vi "set--uid--tags.vi"() -> ()   [LabVIEW 2021]
panel:
  out "Array 2":string[](array[string])
  out "Array":i32[](array[numeric])
  out "error out":errorcluster
  # "String"
  # "Digital"
  # "Multicolumn Listbox"
  # "Digital"
  # "Listbox"
  # "Ring"
  # "Table"
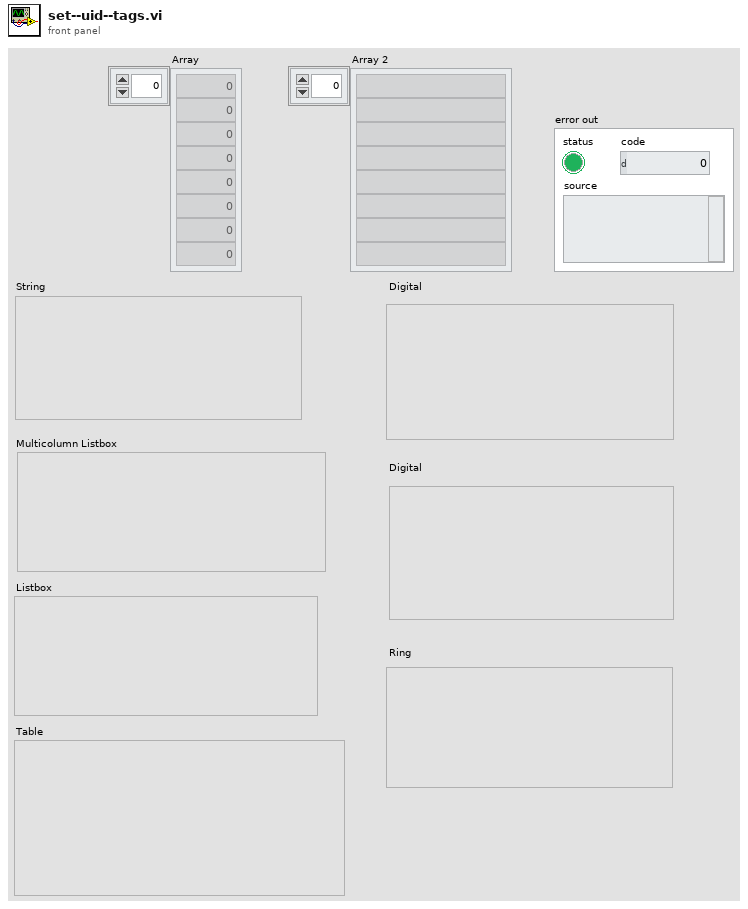
[diagram p1: front panel]
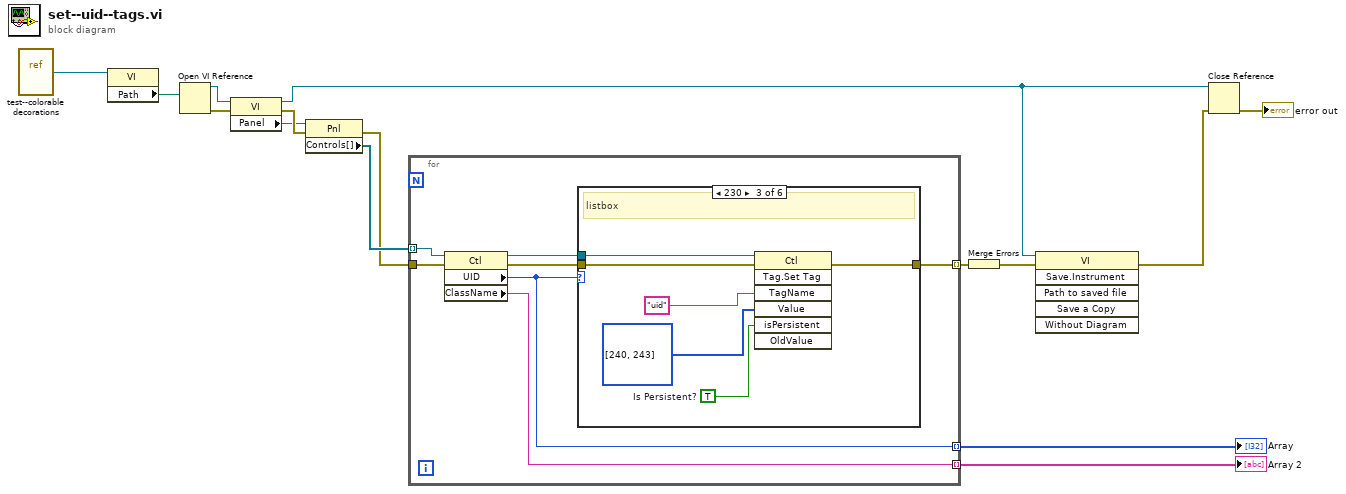
[diagram p0: block diagram]
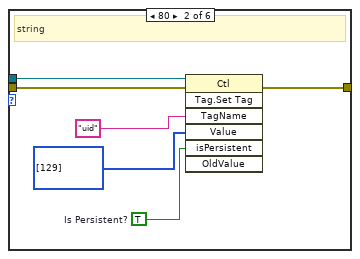
[diagram p3: hidden frame]
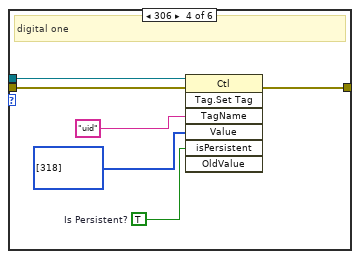
[diagram p4: hidden frame]
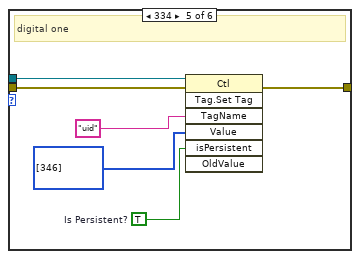
[diagram p5: hidden frame]
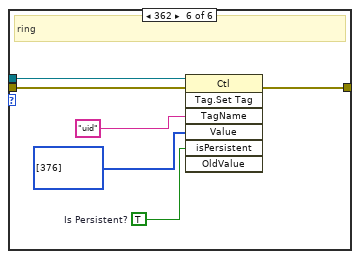
[diagram p6: hidden frame]
diagram:
  n1 = vi-ref "test--colorable decorations.vi"() -> (w15:refnum<vi>)
  n2 = property class="VI"(reference=w15) -> ("Path"=w12:path)  [unwired: 1 in, 2 out]
  n3 = Open VI Reference(vi path=w12) -> (vi reference=w10:refnum<vi>, error out=w14:errorcluster)  [unwired: 5 in]
  n4 = property class="VI"(reference=w10, error in=w14) -> (reference out=w1:refnum<vi>, error out=w11:errorcluster, "Panel"=w9:refnum<vi>)
  n5 = property class="Pnl"(reference=w9, error in=w11) -> (error out=w7:errorcluster, "Controls[]"=w8:refnum<vi>[])  [unwired: 1 out]
  n6 = for {
    tunnel: w8 -> [w20] mode=indexing
    tunnel: w7 -> [w22]
    tunnel: [w18] -> w6 mode=indexing
    tunnel: [w16] -> w4 mode=indexing
    tunnel: [w19] -> w3 mode=indexing
    n7 = property class="Ctl"(reference=w20, error in=w22) -> (reference out=w17:refnum<vi>, error out=w21:errorcluster, "UID"=w16:i32, "ClassName"=w19:string)
    n8 = case shown="230" w16 {
      tunnel: w21 -> [w23 w29 w35 w41 w47 w53]
      tunnel: [w23 w28 w34 w40 w46 w52] -> w18
      tunnel: w17 -> [_ w27 w33 w39 w45 w51]
      frame 0, Default {
      }
      frame 80 {
        w24 = TRUE  # Is Persistent?
        # "string"
        n9 = invoke class="Ctl" method="Tag.Set Tag"(reference=w27, error in=w29, "TagName"="uid" ("Tag Name"), "Value"=i32[] [129], "isPersistent"=w24) -> (error out=w28:errorcluster)  [unwired: 2 in, 6 out]
      }
      frame 230 {
        w30 = TRUE  # Is Persistent?
        # "listbox"
        n10 = invoke class="Ctl" method="Tag.Set Tag"(reference=w33, error in=w35, "TagName"="uid" ("Tag Name"), "Value"=i32[] [240, 243], "isPersistent"=w30) -> (error out=w34:errorcluster)  [unwired: 2 in, 6 out]
      }
      frame 306 {
        w36 = TRUE  # Is Persistent?
        # "digital one"
        n11 = invoke class="Ctl" method="Tag.Set Tag"(reference=w39, error in=w41, "TagName"="uid" ("Tag Name"), "Value"=i32[] [318], "isPersistent"=w36) -> (error out=w40:errorcluster)  [unwired: 2 in, 6 out]
      }
      frame 334 {
        w42 = TRUE  # Is Persistent?
        # "digital one"
        n12 = invoke class="Ctl" method="Tag.Set Tag"(reference=w45, error in=w47, "TagName"="uid" ("Tag Name"), "Value"=i32[] [346], "isPersistent"=w42) -> (error out=w46:errorcluster)  [unwired: 2 in, 6 out]
      }
      frame 362 {
        w48 = TRUE  # Is Persistent?
        # "ring"
        n13 = invoke class="Ctl" method="Tag.Set Tag"(reference=w51, error in=w53, "TagName"="uid" ("Tag Name"), "Value"=i32[] [376], "isPersistent"=w48) -> (error out=w52:errorcluster)  [unwired: 2 in, 6 out]
      }
    }
  }
  "Array" <- w4
  "Array 2" <- w3
  n14 = Merge Errors(w6) -> (w5:errorcluster)
  n15 = invoke class="VI" method="Save.Instrument"(reference=w1, error in=w5) -> (error out=w2:errorcluster)  [unwired: 4 in, 5 out]
  n16 = Close Reference(reference=w1, error in (no error)=w2) -> (error out=→"error out":errorcluster)
